vi "TX Timeout.vi"(8 "error in (no error)":errorcluster, 11 "XNET_CAN_RW in":refnum<class "XNET CAN RW.lvclass">) -> (0 "error out":errorcluster, 2 "ACK Errors":u32)   [LabVIEW 2021, in "XNET CAN RW.lvclass"]
uses:
  XNET CAN RW.lvclass
  C:/Program Files/National Instruments/LabVIEW 2021/vi.lib/CIF Foundation/CIF CAN RW Core/CAN_RW_CORE.lvclass
  <vilib>/CIF Foundation/CIF CAN RW Core/CAN_RW_CORE.lvclass/CAN_RW_CORE.ctl
  typedef/Errors.ctl
  XNET CAN RW.lvclass/XNET CAN RW.ctl
  <vilib>/CIF Foundation/CIF CAN RW Core/Accessors/Read One Shot TX.vi
  Add Error Core.vi
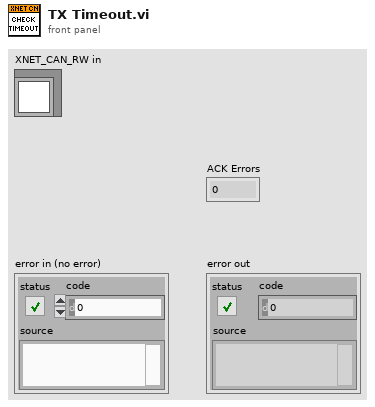
[diagram p1: front panel]
types:
  T1 = typedef "XNET CAN RW.lvclass/Errors.ctl" = enum16{"TX Timeout", "Packet Length", "Invalid Start Time", "Bus Fault"}
  T2 = typedef "CAN_RW_CORE.lvclass/CAN Status.ctl" = cluster{"Comm State":T3, "Last Error":T4, "RX Error Counter":u8, "TX Error Counter":u8}
  T3 = typedef "CAN_RW_CORE.lvclass/Communication State.ctl" = enum16{"Error Active", "Error Passive", "Bus Off"}
  T4 = typedef "CAN_RW_CORE.lvclass/Last Error.ctl" = enum16{"None", "Stuff", "Form", "Ack", "Bit1", "Bit0", "CRC", "Unknown"}
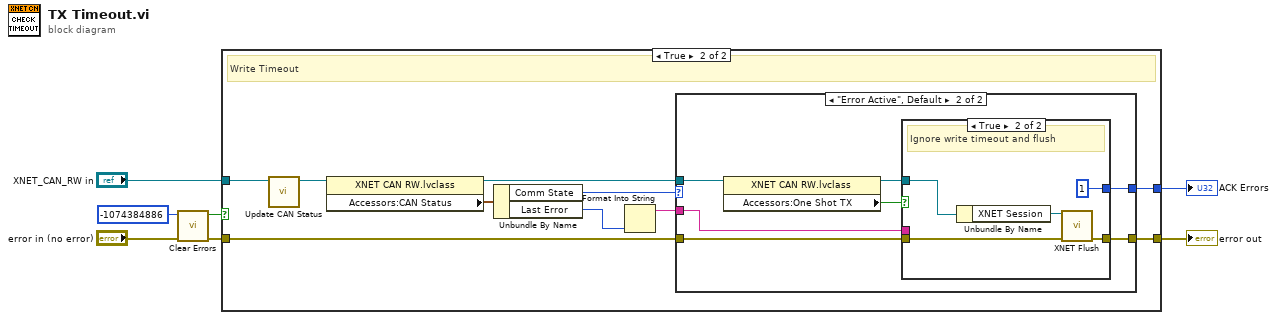
[diagram p0: block diagram]
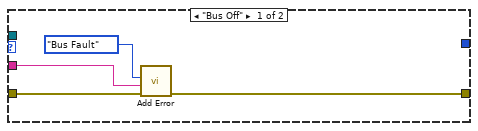
[diagram p3: hidden frame]
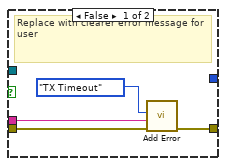
[diagram p4: hidden frame]
diagram:
  n1 = call <vilib>:"Clear Errors.vi"("error in (no error)"="error in (no error)", "specific error code to clear (0: all)"=-1074384886) -> ("error out"=w5:errorcluster, "specific error cleared?"=w3:bool)  [unwired: 4 in]
  n2 = case shown="True" w3 {
    tunnel: w5 -> [w8 w18]
    tunnel: [w8 w17] -> w4
    tunnel: "XNET_CAN_RW in" -> [_ w13]
    tunnel: [_ w16] -> w1
    frame False {
      # "Not write timeout"
    }
    frame True {
      # "Write Timeout"
      n3 = call "Update CAN Status.vi"("XNET CAN RW in"=w13) -> ("XNET CAN RW out"=w15:refnum<class "XNET CAN RW.lvclass">)  [unwired: 9 in, 1 out]
      n4 = property class="XNET CAN RW.lvclass"(reference=w15) -> (reference out=w9:refnum<class "XNET CAN RW.lvclass">, "Accessors:CAN Status"=w14:T2)  [unwired: 1 in, 1 out]
      n5 = Unbundle By Name(w14) -> ("Comm State"=w12:T3, "Last Error"=w11:T4)
      n6 = Format Into String(w11) -> (resulting string=w10:string)  [unwired: 3 in, 1 out]
      n7 = case shown="\"Error Active\", Default" w12 {
        tunnel: w18 -> [w19 w29]
        tunnel: [w21 w28] -> w17
        tunnel: [_ w25] -> w16
        tunnel: w10 -> [w20 w23]
        tunnel: w9 -> [_ w24]
        frame "Bus Off" {
          n8 = call "Add Error.vi"("error in (no error)"=w19, "String to Append"=w20, "Error"=Errors."Bus Fault") -> ("error out"=w21:errorcluster)  [unwired: 8 in]
        }
        frame "Error Active", Default {
          n9 = property class="XNET CAN RW.lvclass"(reference=w24) -> (reference out=w26:refnum<class "XNET CAN RW.lvclass">, "Accessors:One Shot TX"=w27:bool)  [unwired: 1 in, 1 out]
          n10 = case shown="True" w27 {
            tunnel: w29 -> [w31 w37]
            tunnel: [w33 w36] -> w28
            tunnel: w26 -> [_ w35]
            tunnel: [_ u32 1 ("ACK Errors")] -> w25
            tunnel: w23 -> [w30 _]
            frame False {
              # "Replace with clearer error message for user"
              n11 = call "Add Error.vi"("error in (no error)"=w31, "String to Append"=w30, "Error"=Errors."TX Timeout") -> ("error out"=w33:errorcluster)  [unwired: 8 in]
            }
            frame True {
              # "Ignore write timeout and flush"
              n12 = Unbundle By Name(w35) -> ("XNET Session"=w38:refnum<k21>)
              n13 = call <vilib>:"XNET Flush.vi"("session in"=w38, "error in (no error)"=w37) -> ("error out"=w36:errorcluster)  [unwired: 12 in, 1 out]
            }
          }
        }
      }
    }
  }
  "error out" <- w4
  "ACK Errors" <- w1
